vi "Extend Log Path.vi"(10 "logger name":string, 11 "File Handler in":refnum<class "File Handler.lvclass">) -> (3 "File Handler out":refnum<class "File Handler.lvclass">)   [LabVIEW 2018, in "GLog.lvlib" / "File Handler.lvclass"]
uses:
  File Handler.lvclass
  File Handler.lvclass/File Handler.ctl
panel:
  # "Connector Pane"
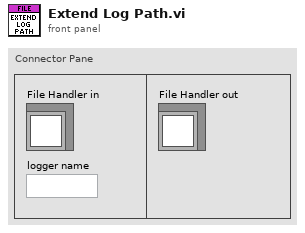
[diagram p1: front panel]
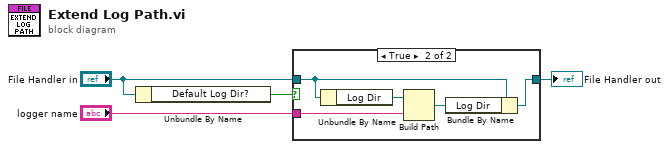
[diagram p0: block diagram]
diagram:
  n1 = Unbundle By Name("File Handler in") -> ("Default Log Dir?"=w1:bool)
  n2 = case shown="True" w1 {
    tunnel: [w5 w9] -> w4
    tunnel: "logger name" -> [_ w8]
    tunnel: "File Handler in" -> [w5 w6]
    frame False {
    }
    frame True {
      n3 = Unbundle By Name(w6) -> ("Log Dir"=w7:path)
      n4 = Build Path(base path=w7, name or relative path=w8) -> (appended path=w10:path)
      n5 = Bundle By Name(cluster=w6, "Log Dir"=w10) -> (w9:refnum<class "File Handler.lvclass">)
    }
  }
  "File Handler out" <- w4
